vi "Example - Screenshot Capture.vi"(8 "error in":errorcluster, 10 "Base File Name (*.bmp)":string="InstrStudio_Screenshot.bmp", 11 "Output Folder to Save Screenshot":path=path "C:/Temp") -> (0 "error out":errorcluster, 3 "Save Image Successful?":bool)   [LabVIEW 2025]
doc: "This example demonstrates how to use the LabVIEW Screenshot Utility VI to capture the InstrumentStudio window.\n\n • Set the output folder and base file name.\n • Ensure InstrumentStudio is running with required SFPs loaded.\n • Run the VI to capture and save the screenshot with a timestamp.\n • Verify the saved image in the specified output folder.\n • Refer to the main VI for additional details and configuration."
uses:
  Screenshot Utility.lvlib
panel:
  # "This example demonstrates basic usage of the LabVIEW Screenshot Utility VI.\n\n • This VI directly calls the main screenshot utility with sample inputs.\n • Configure the output folder and base file name as needed.\n • Ensure InstrumentStudio is running with required SFPs loaded.\n • Run the VI to capture and save the screenshot.\n • Refer to the main VI for detailed functionality and configuration."
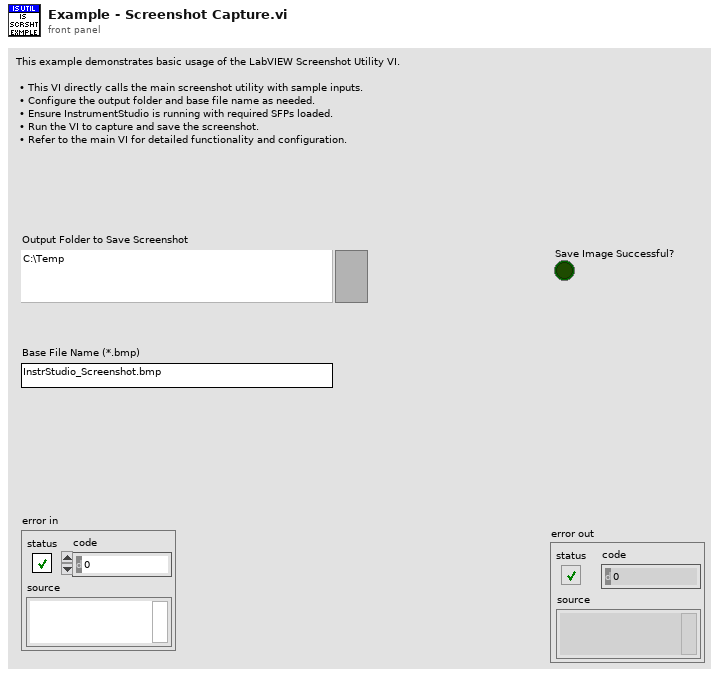
[diagram p1: front panel]
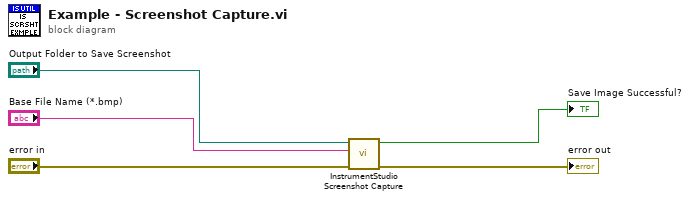
[diagram p0: block diagram]
diagram:
  n1 = call "InstrumentStudio Screenshot Capture.vi"("error in"="error in", "Base File Name (*.bmp)"="Base File Name (*.bmp)", "Output Folder to Save Screenshot"="Output Folder to Save Screenshot") -> ("error out"=→"error out":errorcluster, "Save Image Successful?"=→"Save Image Successful?":bool)  [unwired: 7 in]
